vi "GetAllItemsFromXMLFile.vi"() -> (1 "Mode XML Elements":string, 3 "Array":refnum<class "Link.lvclass">[](array[class]))   [LabVIEW 2023, in "GettingStartedWindow.lvlib"]
uses:
  <resource>/modes/FRC/GSW/GettingStartedWindow.lvlib
  <resource>/modes/FRC/GSW/Classes/Link/Link.lvclass
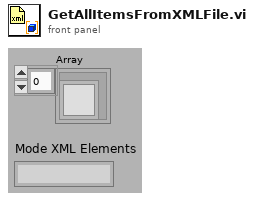
[diagram p1: front panel]
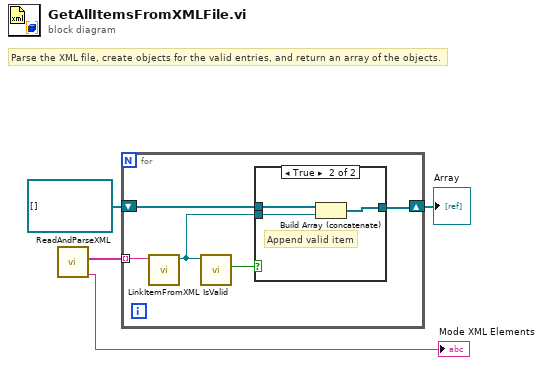
[diagram p0: block diagram]
diagram:
  # "Parse the XML file, create objects for the valid entries, and return an array of the objects."
  n1 = call <resource>:"ReadAndParseXML.vi"() -> ("Mode XML Elements"=→"Mode XML Elements":string, "XML Elements"=w4:string[])  [unwired: 10 out]
  n2 = for {
    tunnel: w4 -> [w9] mode=indexing
    shift-right: [w7] -> w3
    shift-left: refnum<class "Link.lvclass">[] [] -> [w8]
    n3 = call <resource>:"LinkItemFromXML.vi"("XML for one item"=w9) -> ("GettingStartedWindow.lvlib:Link.lvclass"=w6:refnum<class "Link.lvclass">)  [unwired: 10 out]
    n4 = call <resource>:"IsValid.vi"("Link in"=w6) -> ("valid"=w5:bool)  [unwired: 1 in, 9 out]
    n5 = case shown="True" w5 {
      tunnel: w8 -> [w10 w13]
      tunnel: [w10 w12] -> w7
      tunnel: w6 -> [_ w11]
      frame False {
        # "Skip invalid item."
      }
      frame True {
        # "Append valid item"
        n6 = Build Array (concatenate)(w13, w11) -> (w12:refnum<class "Link.lvclass">[])
      }
    }
  }
  "Array" <- w3
